vi "SetPosition.vi"(8 "error in (no error)":errorcluster, 10 "Window Position":cluster{"x":i32, "y":i32}, 11 "Window in":refnum<class "Window.lvclass">) -> (0 "error out":errorcluster, 3 "Window out":refnum<class "Window.lvclass">)   [LabVIEW 2020, in "GLF.lvlib" / "Window.lvclass"]
uses:
  Window.lvclass
  Window.lvclass/Window.ctl
  <vilib>/Saukko/LV SDL3/Sources/SDL3/Video/Video.lvlib
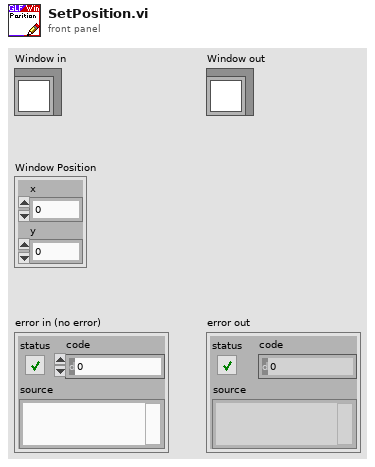
[diagram p1: front panel]
types:
  T1 = typedef "SDL3.lvlib/Video.lvlib/SDL_Window--pointer.ctl" = i64
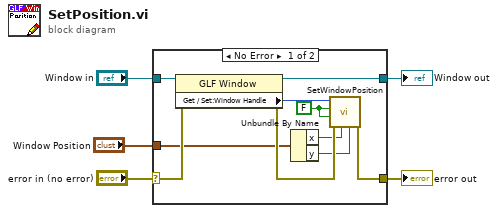
[diagram p0: block diagram]
diagram:
  n1 = case shown="No Error" "error in (no error)" {
    selector: "error in (no error)" -> [w11 w16]
    tunnel: "Window in" -> [w13 w17]
    tunnel: [w14 w16] -> w3
    tunnel: [w12 w17] -> w2
    tunnel: "Window Position" -> [w8 _]
    frame No Error {
      w9 = FALSE ("Center x")
      n2 = property class="GLF Window"(reference=w13, error in=w11) -> (reference out=w12:refnum<class "Window.lvclass">, error out=w15:errorcluster, "Get / Set:Window Handle"=w10:T1)
      n3 = Unbundle By Name(w8) -> ("x"=w7:i32, "y"=w6:i32)
      n4 = call <vilib>:"SetWindowPosition.vi"("y"=w6, "x"=w7, "No Error"=w15, "Center y"=w9, "Center x"=w9, "Window [SDL_Window *]"=w10) -> ("Error Out"=w14:errorcluster)  [unwired: 5 in]
    }
    frame Error {
    }
  }
  "Window out" <- w2
  "error out" <- w3
